vi "Wait.vi"(8 "error in (no error)":errorcluster caption="错误输入（无错误）", 10 "秒":dbl, 11 "LabVIEW对象 2":refnum<class>) -> (0 "error out":errorcluster caption="错误输出", 3 "LabVIEW对象":refnum<class>)   [LabVIEW 2020, in "Data Viewer.lvlib" / "Data Viewer.lvclass"]
uses:
  Data Viewer.lvclass
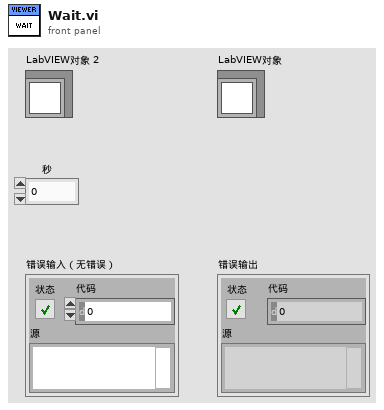
[diagram p1: front panel]
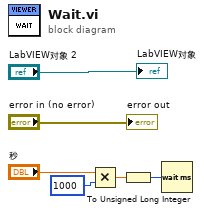
[diagram p0: block diagram]
diagram:
  n1 = Multiply(x="秒", y=1000) -> (x*y=w4:dbl)
  n2 = To Unsigned Long Integer(number=w4) -> (unsigned 32bit integer=w3:u32)
  n3 = Wait (ms)(milliseconds to wait=w3) -> ()  [unwired: 1 out]
  "error out" <- "error in (no error)"
  "LabVIEW对象" <- "LabVIEW对象 2"
